vi "Transport_Receive_Event.vi"(8 "error in (no error)":errorcluster={"status"=FALSE, "code"=0, "source"="\"\""}, 10 "run version":string, 11 "Transport ref":string) -> (0 "error out":errorcluster={"status"=FALSE, "code"=0, "source"="\"\""}, 2 "status ok":bool, 3 "EventRecord":string)   [LabVIEW 2026]
doc: "INTENT: Receive event/status streams. LOGIC: Receive and validate event ordering, detect duplicates, forward to Host state updater."
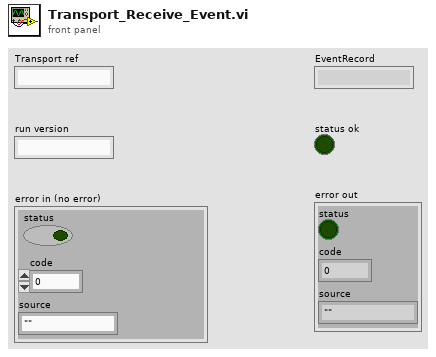
[diagram p1: front panel]
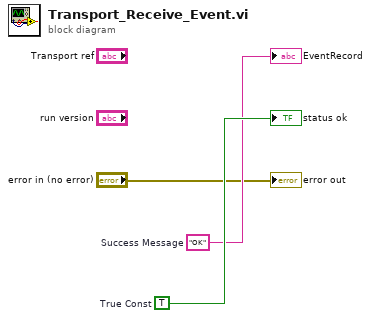
[diagram p0: block diagram]
diagram:
  w3 = TRUE  # True Const
  w2 = "OK"  # Success Message
  "EventRecord" <- w2
  "status ok" <- w3
  "error out" <- "error in (no error)"
